vi "Deserialize CD XML FIle.vi"(8 "Error In":errorcluster caption="error in", 11 "XML Path":path) -> (0 "Error Out":errorcluster caption="error in", 3 "Custom Device .NET Ref Out":refnum<k24>)   [LabVIEW 2015, in "VeriStand Custom Device XML Parser.lvlib"]
doc: "Deserializes the provided custom device XML file and returns a reference to the file in memory."
uses:
  VeriStand Custom Device XML Parser.lvlib
  NationalInstruments.VeriStand.XMLReader
  <vilib>/Utility/sysdir.llb/System Directory Type.ctl
  subVI/Global Settings.vi
  Configuration Tool.lvlib
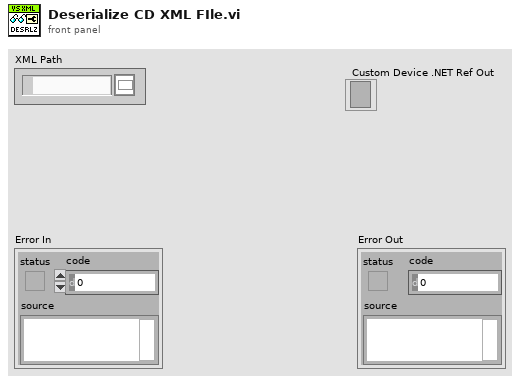
[diagram p1: front panel]
types:
  T1 = typedef "System Directory Type.ctl" = i32
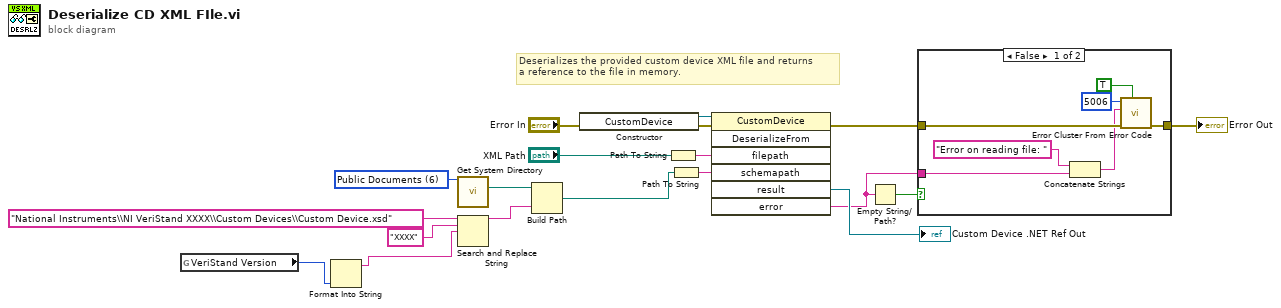
[diagram p0: block diagram]
diagram:
  w15 = T1 6 items=["User Home"=0, "User Desktop"=1, "User Documents"=2, "User Application Data"=3, "User Preferences"=4, "User Temporary"=5, "Public Documents"=6, "Public Application Data"=7, "Public Preferences"=8, "Public Cache"=13, "System Core Libraries"=9, "System Installed Libraries"=10, "Application Files"=11, "Boot Volume Root"=12] ("system directory type")
  # "Deserializes the provided custom device XML file and returns\na reference to the file in memory."
  n1 = global read "Global Settings.vi" "VeriStand Version"() -> (w2:enum16{"2013", "2014", "2015", "2016"})
  n2 = Format Into String(w2) -> (resulting string=w1:string)  [unwired: 3 in, 1 out]
  n3 = call <vilib>:"Get System Directory.vi"("system directory type"=w15) -> ("system directory"=w14:path)  [unwired: 10 in]
  n4 = Search and Replace String(input string="National Instruments\\NI VeriStand XXXX\\Custom Devices\\Custom Device.xsd", search string="XXXX", replace string=w1) -> (result string=w9:string)  [unwired: 5 in, 3 out]
  n5 = Build Path(base path=w14, name or relative path=w9) -> (appended path=w13:path)
  n6 = constructor class="CustomDevice"(error in="Error In") -> (reference out=w17:refnum<k24>, error out=w7:errorcluster)  [unwired: 2 in, 1 out]
  n7 = Path To String(path="XML Path") -> (string=w16:string)
  n8 = Path To String(path=w13) -> (string=w12:string)
  n9 = invoke class="CustomDevice" method="DeserializeFrom"(reference=w17, error in=w7, "filepath"=w16, "schemapath"=w12) -> (error out=w4:errorcluster, "result"=→"Custom Device .NET Ref Out":refnum<k24>, "error"=w5:string)  [unwired: 3 in, 4 out]
  n10 = Empty String/Path?(string/path=w5) -> (empty?=w6:bool)
  n11 = case shown="False" w6 {
    tunnel: w5 -> [w25 _]
    tunnel: w4 -> [w24 w27]
    tunnel: [w21 w27] -> w3
    frame False {
      n12 = Concatenate Strings("Error on reading file: " ("string"), w25) -> (w22:string)
      n13 = call <vilib>:"Error Cluster From Error Code.vi"("show call chain? (False)"=TRUE, "error in (no error)"=w24, "error message (\"\")"=w22, "error code (0)"=5006) -> ("error out"=w21:errorcluster)  [unwired: 5 in]
    }
    frame True {
    }
  }
  "Error Out" <- w3
